vi "Test Deserialize Clusters.vi"(8 "error in (no error)":errorcluster) -> (0 "error out":errorcluster)   [LabVIEW 2013]
uses:
  src/Serializer/JSON Serializer/JSON Serializer.lvclass
  src/Deserializer/JSON Deserializer/JSON Deserializer.lvclass
  src/Library/Empty Cluster.vi
  <userlib>/_OpenG.lib/lvdata/lvdata.llb/Array of VData to VCluster__ogtk.vi
  <vilib>/addons/_JKI Toolkits/Caraya/classes/Test/Test.lvclass
  <vilib>/addons/_JKI Toolkits/Caraya/classes/Assert/Assert.lvclass
  src/JKI JSON Serialization.lvlib
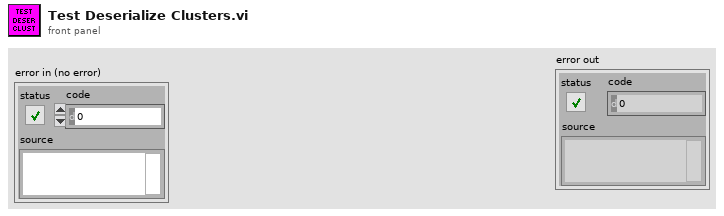
[diagram p1: front panel]
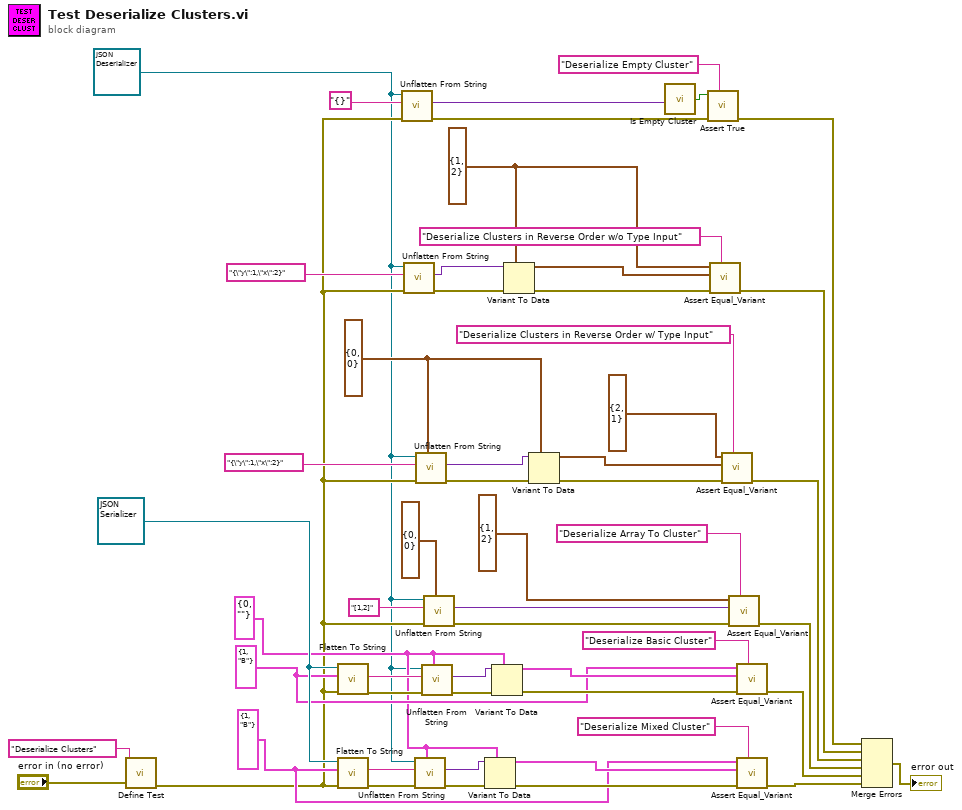
[diagram p0: block diagram]
diagram:
  w19 = cluster{"x":i32, "y":i32} {"x"=1, "y"=2}
  w12 = cluster{"x":i32, "y":i32} {"x"=0, "y"=0}
  w26 = cluster{"a":i32, "b":string} {"a"=0, "b"=""}
  w37 = cluster{"a":i32, string} {"a"=1, "B"}
  w28 = cluster{"a":i32, "b":string} {"a"=1, "b"="B"}
  w5 = refnum<class "JSON Deserializer.lvclass"> refnum ("Deserializer in")
  w36 = refnum<class "JSON Serializer.lvclass"> refnum ("JKI JSON Serialization.lvlib:JSON Serializer.lvclass")
  n1 = call <vilib>:"Define Test.vi"("error in (no error)"="error in (no error)", "Label (VI Title)"="Deserialize Clusters") -> ("error out"=w6:errorcluster)  [unwired: 9 in]
  n2 = call-dynamic "Flatten To String.vi"("error in (no error)"=w6, "Variant"=w28, "JSON Serializer in"=w36) -> ("error out"=w48:errorcluster, "String"=w47:string)  [unwired: 6 in, 1 out]
  n3 = call-dynamic "Flatten To String.vi"("error in (no error)"=w6, "Variant"=w37, "JSON Serializer in"=w36) -> ("error out"=w41:errorcluster, "String"=w40:string)  [unwired: 6 in, 1 out]
  n4 = call-dynamic "Unflatten From String.vi"("error in (no error)"=w6, "String"="{}", "Deserializer in"=w5) -> ("error out"=w4:errorcluster, "Variant"=w3:variant)  [unwired: 6 in, 1 out]
  n5 = call-dynamic "Unflatten From String.vi"("error in (no error)"=w6, "String"="{\"y\":1,\"x\":2}", "Deserializer in"=w5) -> ("error out"=w21:errorcluster, "Variant"=w20:variant)  [unwired: 6 in, 1 out]
  n6 = call-dynamic "Unflatten From String.vi"("Type and Defaults"=w26, "error in (no error)"=w41, "String"=w40, "Deserializer in"=w5) -> ("error out"=w43:errorcluster, "Variant"=w42:variant)  [unwired: 5 in, 1 out]
  n7 = call-dynamic "Unflatten From String.vi"("Type and Defaults"=w12, "error in (no error)"=w6, "String"="{\"y\":1,\"x\":2}", "Deserializer in"=w5) -> ("error out"=w10:errorcluster, "Variant"=w11:variant)  [unwired: 5 in, 1 out]
  n8 = call-dynamic "Unflatten From String.vi"("Type and Defaults"=w26, "error in (no error)"=w48, "String"=w47, "Deserializer in"=w5) -> ("error out"=w46:errorcluster, "Variant"=w27:variant)  [unwired: 5 in, 1 out]
  n9 = call-dynamic "Unflatten From String.vi"("Type and Defaults"=cluster{"x":i32, "y":i32} {"x"=0, "y"=0}, "error in (no error)"=w6, "String"="[1,2]", "Deserializer in"=w5) -> ("error out"=w31:errorcluster, "Variant"=w30:variant)  [unwired: 5 in, 1 out]
  n10 = Variant To Data(error in=w43, type=w26, Variant=w42) -> (data=w38:cluster{"a":i32, "b":string}, error out=w39:errorcluster)
  n11 = Variant To Data(error in=w46, type=w26, Variant=w27) -> (data=w45:cluster{"a":i32, "b":string}, error out=w44:errorcluster)
  n12 = Variant To Data(error in=w21, type=w19, Variant=w20) -> (data=w17:cluster{"x":i32, "y":i32}, error out=w18:errorcluster)
  n13 = Variant To Data(error in=w10, type=w12, Variant=w11) -> (data=w13:cluster{"x":i32, "y":i32}, error out=w9:errorcluster)
  n14 = call "Is Empty Cluster.vi"("Deserialized JSON Data"=w3) -> ("Empty Cluster?"=w2:bool)
  n15 = call <vilib>:"Assert True.vi"("Label"="Deserialize Empty Cluster", "error in (no error)"=w4, "True?"=w2) -> ("error out"=w1:errorcluster)  [unwired: 8 in]
  n16 = call <vilib>:"Assert Equal_Variant.vi"("Label"="Deserialize Clusters in Reverse Order w/o Type Input", "error in (no error)"=w18, "Y"=w17, "X"=w19) -> ("error out"=w22:errorcluster)  [unwired: 7 in]
  n17 = call <vilib>:"Assert Equal_Variant.vi"("Label"="Deserialize Clusters in Reverse Order w/ Type Input", "error in (no error)"=w9, "Y"=w13, "X"=cluster{"x":i32, "y":i32} {"x"=2, "y"=1}) -> ("error out"=w24:errorcluster)  [unwired: 7 in]
  n18 = call <vilib>:"Assert Equal_Variant.vi"("Label"="Deserialize Array To Cluster", "error in (no error)"=w31, "Y"=w30, "X"=cluster{"x":i32, "y":i32} {"x"=1, "y"=2}) -> ("error out"=w32:errorcluster)  [unwired: 7 in]
  n19 = call <vilib>:"Assert Equal_Variant.vi"("Label"="Deserialize Basic Cluster", "error in (no error)"=w44, "Y"=w45, "X"=w28) -> ("error out"=w50:errorcluster)  [unwired: 7 in]
  n20 = call <vilib>:"Assert Equal_Variant.vi"("Label"="Deserialize Mixed Cluster", "error in (no error)"=w39, "Y"=w38, "X"=w37) -> ("error out"=w51:errorcluster)  [unwired: 7 in]
  n21 = Merge Errors(w1, w22, w24, w32, w50, w51) -> (→"error out":errorcluster)
